vi "fix_shared_library_paths_for_package.vi"(8 "error in":errorcluster, 11 "Package File Path":path) -> (0 "error out":errorcluster)   [LabVIEW 2020]
uses:
  Package/PackageFile.lvclass
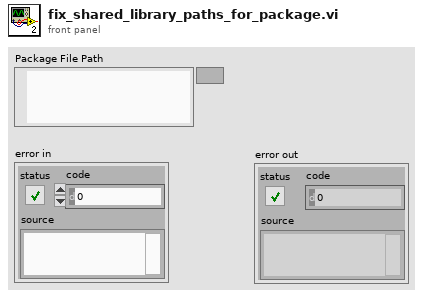
[diagram p1: front panel]
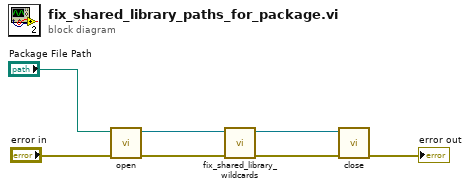
[diagram p0: block diagram]
diagram:
  n1 = call "open.vi"("error in"="error in", "Package File Path"="Package File Path") -> ("error out"=w4:errorcluster, "PackageFile out"=w3:refnum<class "PackageFile.lvclass">)  [unwired: 8 in]
  n2 = call "fix_shared_library_wildcards.vi"("error in (no error)"=w4, "UnpackedPackage in"=w3) -> ("error out"=w2:errorcluster, "UnpackedPackage out"=w1:refnum<class "PackageFile.lvclass">)  [unwired: 7 in, 1 out]
  n3 = call "close.vi"("error in (no error)"=w2, "PackageFile in"=w1) -> ("error out"=→"error out":errorcluster)  [unwired: 8 in, 1 out]
